vi "OverlayPoint.vi"(6 "Color":u32(colorbox)=16711680, 7 "GroupName":string, 8 "error in":errorcluster, 10 "Point":T1, 11 "Image Reference In":T2) -> (0 "error out":errorcluster, 3 "Image Reference Out":T2)   [LabVIEW 2020, in "OpenLvVision_Overlays.lvlib"]
doc: "Overlays a point on top of an image."
uses:
  OpenLvVision_Overlays.lvlib
  <vilib>/OpenLvVision/OpenLvVision_Image/Management/TypeDef/OLV Image.ctl
  TypeDefs/PointI32.ctl
  <vilib>/OpenLvVision/OpenLvVision_Image/Management/OLV Management.lvlib
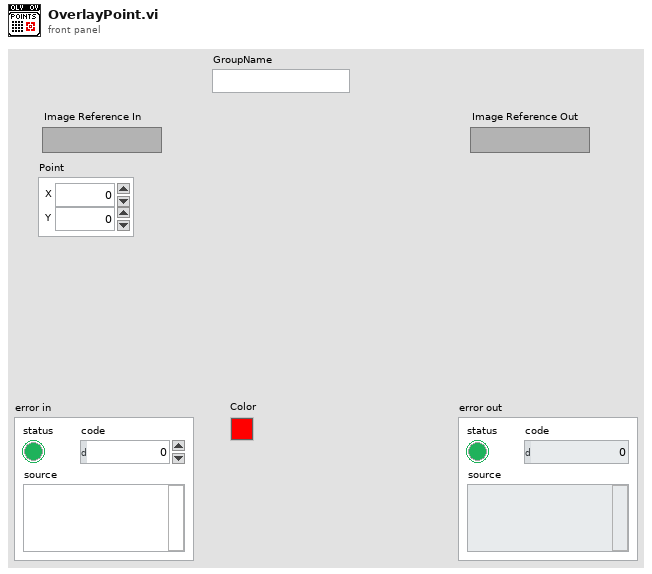
[diagram p1: front panel]
types:
  T1 = typedef "OpenLvVision_Overlays.lvlib/PointI32.ctl" = cluster{"X":i32, "Y":i32}
  T2 = typedef "OLV OpenLvVision_Image.lvlib/OLV Management.lvlib/OLV Image.ctl" = refnum<image>
  T3 = typedef "IMAQ Image.ctl" = refnum<image>
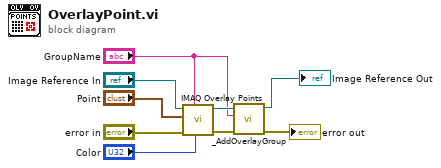
[diagram p0: block diagram]
diagram:
  n1 = call "IMAQ Overlay Points"("Color"="Color", "Group"="GroupName", "error in (no error)"="error in", "Point"="Point", "Image"="Image Reference In") -> ("error out"=w4:errorcluster, "Image Out"=w5:T3)  [unwired: 5 in]
  n2 = call "_AddOverlayGroup.vi"("error in"=w4, "GroupName"="GroupName", "Image Reference In"=w5) -> ("error out"=→"error out":errorcluster, "Image Reference Out"=→"Image Reference Out":T2)  [unwired: 7 in]
